vi "IsWindowEnabled Wrapper Template.vi"(0 "hWnd":u64, 11 "error in":errorcluster) -> (4 "enabled?":bool, 15 "error out":errorcluster)   [LabVIEW 2020]
doc: "TRUE when the window hWnd takes mouse and keyboard input, through user32.dll IsWindowEnabled (stdcall, called in any thread). A window behind a modal dialog is disabled - LabVIEW disables every one of its windows while a dialog such as the Two Button Dialog or a file dialog is up (measured on LabVIEW 2025). FALSE also when hWnd is not a window. When error in carries an error the DLL is not called. Generated by tools\\Build Win32 Wrappers.vi - do not edit by hand, rebuild it."
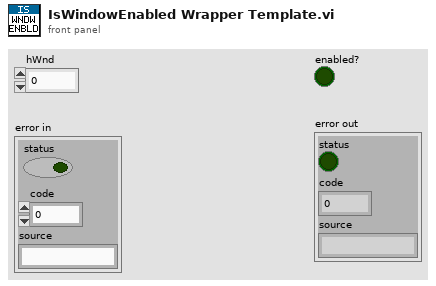
[diagram p1: front panel]
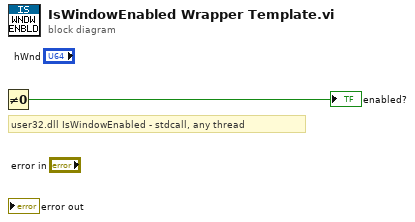
[diagram p0: block diagram]
diagram:
  # "user32.dll IsWindowEnabled - stdcall, any thread"
  n1 = Not Equal To 0?() -> (x != 0?=→"enabled?":bool)  [unwired: 1 in]
